vi "test timestamp to epoch.vi"(8 "error in (no error)":errorcluster, 11 "TestCase in":refnum<class "Timestamp Tests.lvclass">) -> (0 "error out":errorcluster, 3 "TestCase out":refnum<class "Timestamp Tests.lvclass">)   [LabVIEW 2020, in "Timestamp Tests.lvclass"]
uses:
  Timestamp Tests.lvclass
  <vilib>/Utility/file.llb/Application Directory.vi
  <vilib>/Utility/libraryn.llb/Check if File or Folder Exists.vi
  <vilib>/addons/_JKI Toolkits/VI Tester/TestCase.llb/TestCase.lvclass
  C:/Program Files/National Instruments/LabVIEW 2024/vi.lib/addons/_JKI Toolkits/VI Tester/TestCase.llb/TestCase.lvclass
panel:
  out "Returned":string
  out "Expected":string
  out "return type":dbl format="%#_23g"
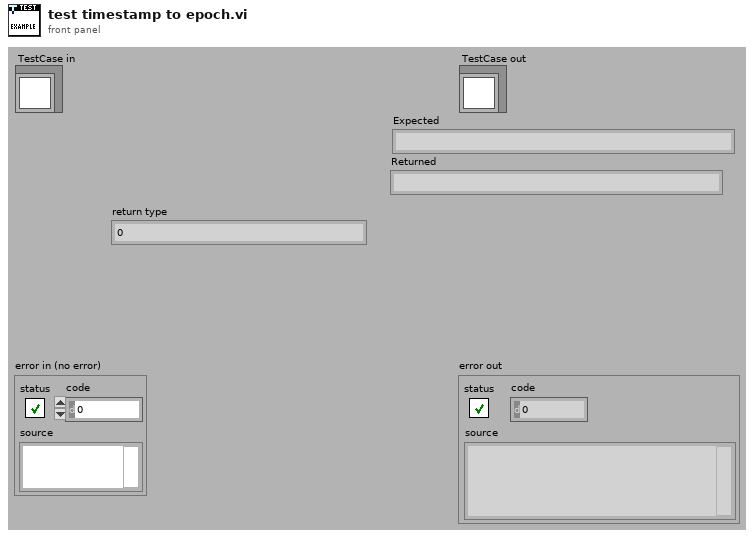
[diagram p1: front panel]
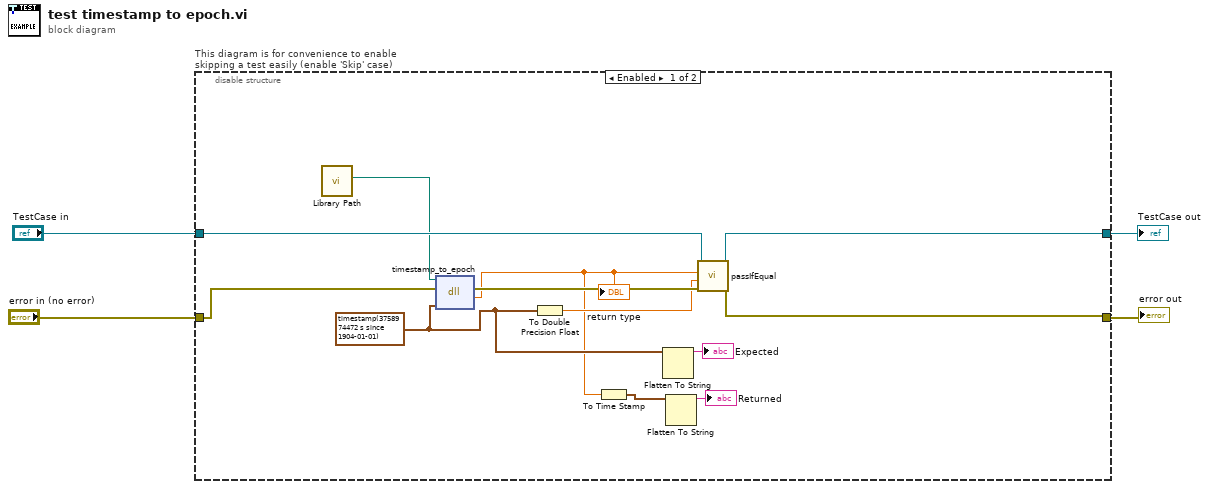
[diagram p0: block diagram]
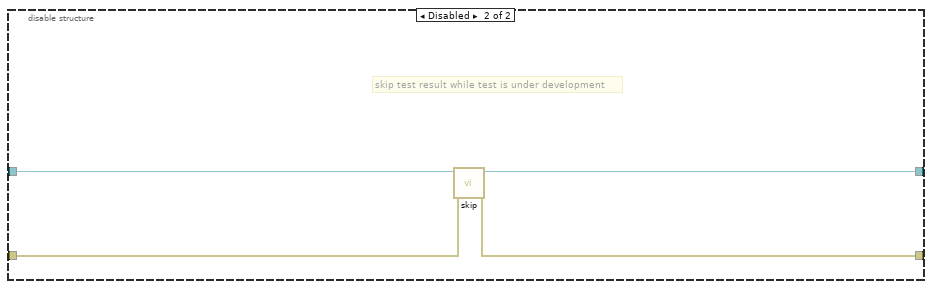
[diagram p2: hidden frame]
diagram:
  n1 = disable-structure "This diagram is for convenience to enable skipping a test easily (enable 'Skip' case)" shown="Enabled" {
    disable-tunnel: "TestCase in" -> [w16 w20]
    disable-tunnel: [w15 w18] -> w1
    disable-tunnel: [w14 w19] -> w3
    disable-tunnel: "error in (no error)" -> [w13 w17]
    frame Enabled {
      w7 = timestamp(3758974472.02441 s since 1904-01-01) ("Time Stamp")
      n2 = call "Library Path.vi"() -> ("Library Path"=w11:path)  [unwired: 11 in]
      n3 = dll-call lib="C:/Users/JamesMcNally/Documents/RustInterop/Rust-LabVIEW-Interop/target/debug/labview_test_library.dll" fn="timestamp_to_epoch"(path in=w11, error in=w13, "timestamp"=w7) -> (error out=w12:errorcluster, "return type"=w6:dbl)  [unwired: 2 in, 1 out]
      "return type" <- w6
      n4 = To Double Precision Float(number=w7) -> (double precision float=w10:dbl)
      n5 = To Time Stamp(1:w6) -> (0:w5:timestamp)
      n6 = Flatten To String(anything=w7) -> (data string=→"Expected":string)  [unwired: 3 in, 2 out]
      n7 = Flatten To String(anything=w5) -> (data string=→"Returned":string)  [unwired: 3 in, 2 out]
      n8 = call-dynamic "passIfEqual.vi"("error in (no error)"=w12, "y"=w10, "x"=w6, "TestCase in"=w16) -> ("error out"=w14:errorcluster, "TestCase out"=w15:refnum<class "Timestamp Tests.lvclass">)  [unwired: 6 in]
    }
    frame Disabled {
      # "skip test result while test is under development"
      n9 = call <vilib>:"skip.vi"("error in (no error)"=w17, "TestCase in"=w20) -> ("error out"=w19:errorcluster, "TestCase out"=w18:refnum<class "Timestamp Tests.lvclass">)  [unwired: 8 in]
    }
  }
  "error out" <- w3
  "TestCase out" <- w1
